vi "TestAccessibilty.vi"(8 "error in":errorcluster) -> (0 "error out":errorcluster)   [LabVIEW 2016, in "WeatherReportTests.lvlib"]
uses:
  WeatherReportTests.lvlib
  APIs/Stimulus/ControlValue/SetValueAuto.vi
  APIs/Stimulus/ControlValue/Controls/Tree/SetValueByHierarchicalPath.vi
  APIs/Stimulus/ControlValue/Controls/Listbox/SetValueByItemName.vi
  APIs/Assert/AssertControlProperty/AssertControlDisable/AssertEnabled.vi
  APIs/Assert/AssertControlProperty/AssertControlDisable/AssertDisabled.vi
  APIs/Assert/AssertControlProperty/AssertControlDisable/AssertDisabledAndGrayedOut.vi
  APIs/Stimulus/VI/CloseVI.vi
  Drona.lvlib
  <vilib>/addons/_JKI Toolkits/Caraya/classes/Test/Test.lvclass
  APIs/Stimulus/ControlValue/Controls/Listbox/StimulusListbox.lvlib
  APIs/Stimulus/VI/VI.lvlib
  APIs/Assert/AssertControlProperty/AssertControlDisable/AssertControlDisable.lvlib
  APIs/Stimulus/ControlValue/Controls/Tree/StimulusTree.lvlib
  APIs/Stimulus/ControlValue/ControlValue.lvlib
panel:
  # "Drona Test Accessibilty"
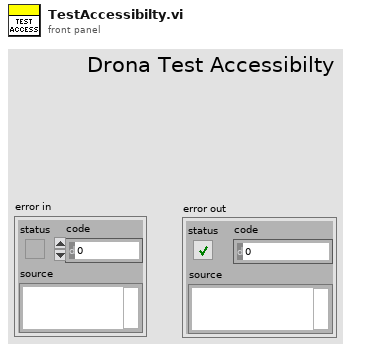
[diagram p1: front panel]
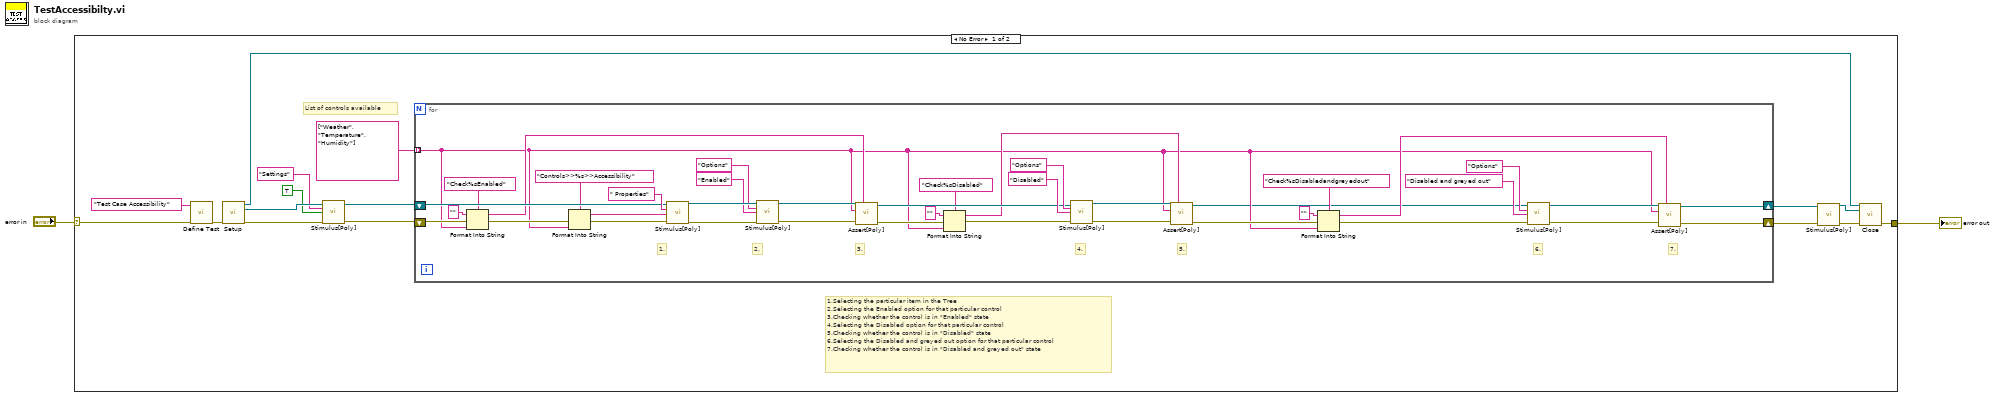
[diagram p0: block diagram]
diagram:
  n1 = case shown="No Error" "error in" {
    selector: "error in" -> [w16 w58]
    tunnel: [w8 w58] -> w1
    frame No Error {
      # "1.Selecting the particular item in the Tree\n2.Selecting the Enabled option for that particular control\n3.Checking whether the control is in \"Enabled\" state\n4.Selecting the Disabled option for that particular control\n5.Checking whether the control is in \"Disabled\" state\n6.Selecting the Disabled and greyed out option for that particular control\n7.Checking whether the control is in \"Disabled and greyed out\" state"
      # "List of controls available"
      n2 = call <vilib>:"Define Test.vi"("error in (no error)"=w16, "Label (VI Title)"="Test Case Accessibility") -> ("error out"=w18:errorcluster)  [unwired: 8 in, 1 out]
      n3 = call "Setup.vi"("error in"=w18) -> ("Application Ref"=w9:refnum<vi>, "VI Reference Out"=w15:refnum<vi>, "error out"=w14:errorcluster)  [unwired: 12 in]
      n4 = call-poly "Stimulus[Poly].vi"("VI Reference In"=w15, "Control Path"="Settings", "Value (Signaling)"=TRUE, "error in"=w14) -> ("VI Reference Out"=w7:refnum<vi>, "error out"=w5:errorcluster)  [unwired: 10 in]
      n5 = for {
        tunnel: string[] ["Weather", "Temperature", "Humidity"] ("Control Path") -> [w21] mode=indexing
        shift-right: [w19] -> w4
        shift-left: w7 -> [w42]
        shift-right: [w40] -> w6
        shift-left: w5 -> [w36]
        # "7."
        # "6."
        # "5."
        # "4."
        # "3."
        # "2."
        # "1."
        n6 = Format Into String(format string="Check%sEnabled" ("Label"), initial string="", error in=w36, w21) -> (resulting string=w33:string, error out=w35:errorcluster)
        n7 = Format Into String(format string="Controls>>%s>>Accessibility" ("Control Path"), error in=w35, w21) -> (resulting string=w38:string, error out=w39:errorcluster)  [unwired: 1 in]
        n8 = call-poly "Stimulus[Poly].vi"("VI Reference In"=w42, "Control Path"=" Properties", "Hierarchical Path"=w38, "Error In"=w39) -> ("VI Reference Out"=w47:refnum<vi>, "Error Out"=w48:errorcluster)  [unwired: 10 in]
        n9 = call-poly "Stimulus[Poly].vi"("VI Reference In"=w47, "Control Path"="Options", "Item Name"="Enabled", "Error In"=w48) -> ("VI Reference Out"=w44:refnum<vi>, "Error Out"=w43:errorcluster)  [unwired: 10 in]
        n10 = call-poly "Assert[Poly].vi"("VI Reference In"=w44, "Test Label"=w33, "Control Path"=w21, "Error In"=w43) -> ("VI Reference Out"=w41:refnum<vi>, "Error Out"=w29:errorcluster)  [unwired: 9 in, 1 out]
        n11 = Format Into String(format string="Check%sDisabled" ("Label"), initial string="", error in=w29, w21) -> (resulting string=w27:string, error out=w28:errorcluster)
        n12 = call-poly "Stimulus[Poly].vi"("VI Reference In"=w41, "Control Path"="Options", "Item Name"="Disabled", "Error In"=w28) -> ("VI Reference Out"=w55:refnum<vi>, "Error Out"=w54:errorcluster)  [unwired: 10 in]
        n13 = call-poly "Assert[Poly].vi"("VI Reference In"=w55, "Test Label"=w27, "Control Path"=w21, "Error In"=w54) -> ("VI Reference Out"=w20:refnum<vi>, "Error Out"=w24:errorcluster)  [unwired: 9 in, 1 out]
        n14 = Format Into String(format string="Check%sDisabledandgreyedout" ("Label"), initial string="", error in=w24, w21) -> (resulting string=w22:string, error out=w23:errorcluster)
        n15 = call-poly "Stimulus[Poly].vi"("VI Reference In"=w20, "Control Path"="Options", "Item Name"="Disabled and greyed out", "Error In"=w23) -> ("VI Reference Out"=w52:refnum<vi>, "Error Out"=w53:errorcluster)  [unwired: 10 in]
        n16 = call-poly "Assert[Poly].vi"("VI Reference In"=w52, "Test Label"=w22, "Control Path"=w21, "Error In"=w53) -> ("VI Reference Out"=w19:refnum<vi>, "Error Out"=w40:errorcluster)  [unwired: 9 in, 1 out]
      }
      n17 = call-poly "Stimulus[Poly].vi"("VI Reference In"=w4, "error in"=w6) -> ("VI Reference Out"=w11:refnum<vi>, "error out"=w10:errorcluster)  [unwired: 12 in]
      n18 = call "Close.vi"("Application Ref"=w9, "VI Reference"=w11, "error in"=w10) -> ("error out"=w8:errorcluster)  [unwired: 12 in]
    }
    frame Error {
    }
  }
  "error out" <- w1
